vi "Multiple Register.vi"() -> ()   [LabVIEW 2018]
uses:
  api/GLog.lvlib
panel:
  out "multiple register test":bool
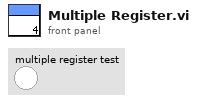
[diagram p1: front panel]
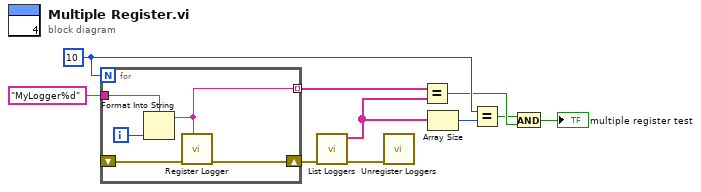
[diagram p0: block diagram]
diagram:
  w9 = 10
  n1 = for {
    N: w9 -> [_]
    tunnel: "MyLogger%d" ("name") -> [w14]
    tunnel: [w13] -> w8 mode=indexing
    shift-right: [w11] -> w2
    shift-left: _ -> [w12]
    i -> [w15]
    n2 = Format Into String(format string=w14, w15) -> (resulting string=w13:string)  [unwired: 2 in, 1 out]
    n3 = call "Register Logger.vi"("name (\"Default\")"=w13, "error in (no error)"=w12) -> ("error out"=w11:errorcluster)  [unwired: 9 in]
  }
  n4 = call "List Loggers.vi"("error in (no error)"=w2) -> ("error out"=w1:errorcluster, "registered loggers"=w7:string[])  [unwired: 9 in]
  n5 = call "Unregister Loggers.vi"("error in (no error)"=w1) -> ()  [unwired: 9 in, 2 out]
  n6 = Equal?(x=w8, y=w7) -> (x = y?=w6:bool)
  n7 = Array Size(array=w7) -> (size(s)=w10:i32)
  n8 = Equal?(x=w9, y=w10) -> (x = y?=w4:bool)
  n9 = And(x=w4, y=w6) -> (x .and. y?=→"multiple register test":bool)
